vi "VIH HelpGen - Write HTML File - Menu - Palette Description.vi"(5 "HTML Folder":path, 6 "Description Params":cluster{"DscrMode":T1, "Description":string}, 7 "Image Folder":path, 8 "error in":errorcluster, 10 "HTML in":string, 11 "Menu Path":path) -> (0 "error out":errorcluster, 2 "HTML out":string, 3 "dup Menu Path":path)   [LabVIEW 2014]
doc: "::: VI Helpeks :::\nCopyright (c) 2000-2026 Konstantin Shifershteyn. All rights reserved."
uses:
  VIH HelpGen Typedef - Enum - Description Mode.ctl
panel:
  # "VI Helpeks\nCopyright (c) 2012-2026 Konstantin Shifershteyn"
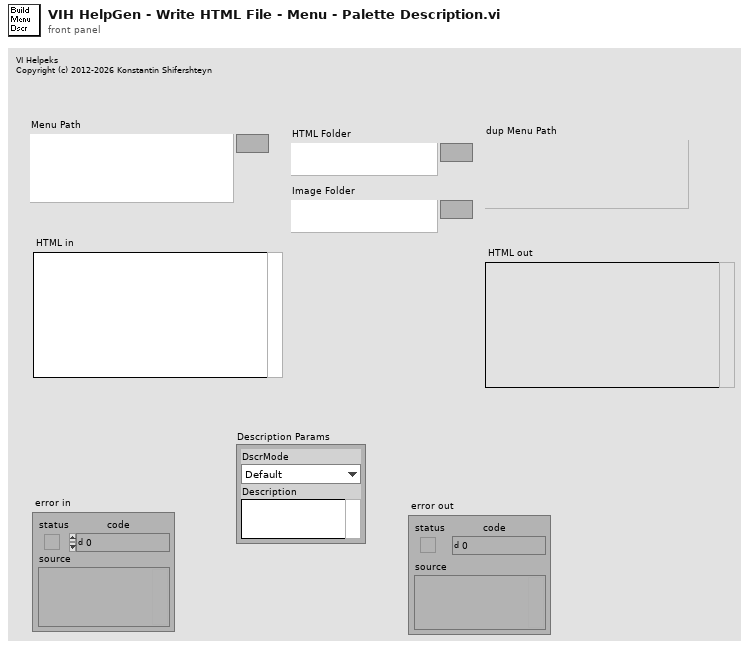
[diagram p1: front panel]
types:
  T1 = typedef "VIH HelpGen Typedef - Enum - Description Mode.ctl" = enum16{"Default", "Description", "Description1", "Description2", "Custom", "None"}
  T2 = typedef "Palette Menu.lvlib/Palette Data.ctl" = cluster{"display name":string, "view format":T3, "palette width":i16, "items":T4, "256 color icon":picture, "B&W color icon":picture, "help information":T6, "palette description":string, "synchronize information":T7}
  T3 = typedef "Palette Menu.lvlib/View Format.ctl" = u16
  T4 = typedef "Palette Menu.lvlib/Items.ctl" = T5[]
  T5 = typedef "Palette Menu.lvlib/Item.ctl" = cluster{"item path":path, "library path (.lvlib)":path, "use default lvlib palette":bool, "short name":string, "place VI contents":bool, "hide synchronized item":bool, "reserve spot for synch item":bool, "configure when placing VI contents":bool}
  T6 = typedef "Palette Menu.lvlib/Help Info.ctl" = cluster{"help tag":string, "help file path ":path}
  T7 = typedef "Palette Menu.lvlib/Synchronize Info.ctl" = cluster{"synchronize with directory":bool, "synchronize directory path":path}
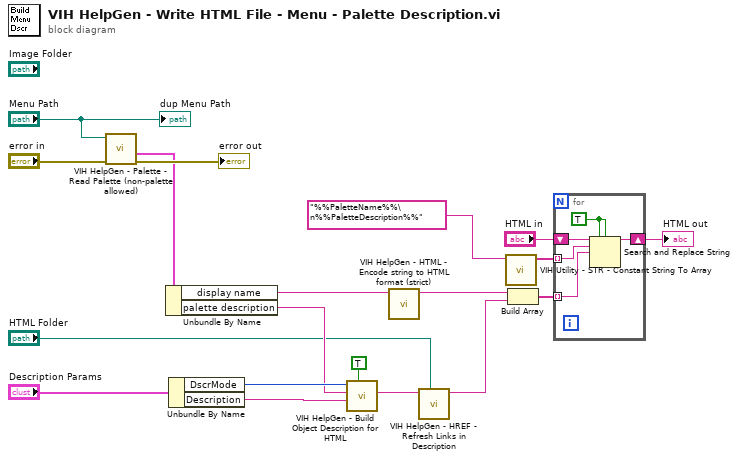
[diagram p0: block diagram]
diagram:
  n1 = call "VIH HelpGen - Palette - Read Palette (non-palette allowed).vi"("error in"="error in", "Palette Path"="Menu Path") -> ("error out"=→"error out":errorcluster, "palette data"=w2:T2)  [unwired: 7 in, 1 out]
  n2 = Unbundle By Name(w2) -> ("display name"=w9:string, "palette description"=w10:string)
  n3 = Unbundle By Name("Description Params") -> ("DscrMode"=w13:T1, "Description"=w14:string)
  n4 = call "VIH HelpGen - Build Object Description for HTML.vi"("Ena \"No Description\" message (F)"=TRUE, "Custom Description"=w14, "Default Description"=w10, "DscrMode"=w13) -> ("Description HTML out"=w7:string)  [unwired: 6 in, 1 out]
  n5 = call "VIH HelpGen - HTML - Encode string to HTML format (strict).vi"("string"=w9) -> ("HTML string"=w8:string)  [unwired: 10 in]
  n6 = call "VIH HelpGen - HREF - Refresh Links in Description.vi"("HTML Folder"="HTML Folder", "Description in"=w7) -> ("Description out"=w6:string)  [unwired: 9 in]
  n7 = call "VIH Utility - STR - Constant String To Array.vi"("String in"="%%PaletteName%%\n%%PaletteDescription%%") -> ("Array out"=w17:string[])  [unwired: 10 in]
  n8 = Build Array(w8, w6) -> (w16:string[])
  n9 = for {
    shift-right: [w23] -> w15
    shift-left: "HTML in" -> [w24]
    tunnel: w17 -> [w21] mode=indexing
    tunnel: w16 -> [w20] mode=indexing
    w22 = TRUE
    n10 = Search and Replace String(replace all?=w22, case sensitive?=w22, input string=w24, search string=w21, replace string=w20) -> (result string=w23:string)  [unwired: 3 in, 3 out]
  }
  "HTML out" <- w15
  "dup Menu Path" <- "Menu Path"
